vi "Get CTRL Area.vi"(6 "SizeOffset (16)":u32=16, 8 "error in (no error)":errorcluster, 9 "Pane in":refnum<vi>, 11 "Control in":refnum<vi>) -> (0 "error out":errorcluster, 1 "Pane out":refnum<vi>, 2 "InsideTheUI":bool, 3 "Control out":refnum<vi>, 5 "CTRL Area":T1)   [LabVIEW 2019, in "Language Editor.lvlib"]
doc: "- - -\nCopyright (c) 2026, Merecs Engineering GmbH"
uses:
  Language Editor.lvlib
panel:
  # "Connector Pane"
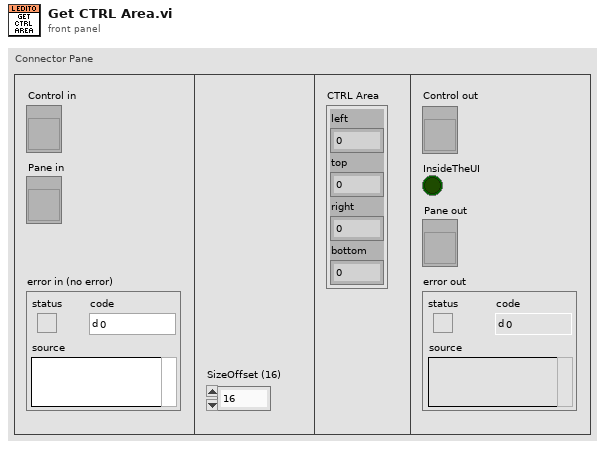
[diagram p1: front panel]
types:
  T1 = cluster{"left":i16, "top":i16, "right":i16, "bottom":i16}
  T2 = typedef "LVPositionTypeDef.ctl" = cluster{"Left":i32, "Top":i32}
  T3 = typedef "LVBoundsTypeDef.ctl" = cluster{"Width":u32, "Height":u32}
  T4 = typedef "LVRectTypeDef.ctl" = cluster{"Left":i16, "Top":i16, "Right":i16, "Bottom":i16}
  T5 = typedef "LVPointTypeDef.ctl" = cluster{"Horizontal":i16, "Vertical":i16}
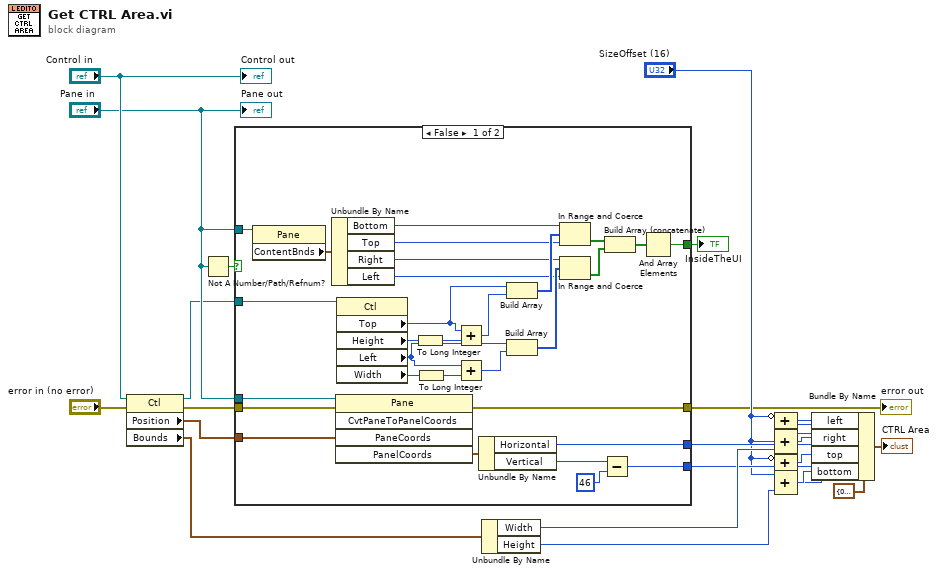
[diagram p0: block diagram]
diagram:
  n1 = property class="Ctl"(reference="Control in", error in="error in (no error)") -> (reference out=w2:refnum<vi>, error out=w10:errorcluster, "Position"=w21:T2, "Bounds"=w9:T3)
  n2 = Not A Number/Path/Refnum?(number/path/refnum="Pane in") -> (NaN/Path/Refnum?=w4:bool)
  n3 = case shown="False" w4 {
    tunnel: w21 -> [w49 _]
    tunnel: "Pane in" -> [w46 _]
    tunnel: w10 -> [w45 w52]
    tunnel: [w44 _] -> w8
    tunnel: [w43 _] -> w7
    tunnel: [w42 w52] -> w5
    tunnel: "Pane in" -> [w22 _]
    tunnel: w2 -> [w37 _]
    tunnel: [w31 _] -> w1
    frame False {
      n4 = property class="Pane"(reference=w22) -> ("ContentBnds"=w27:T4)  [unwired: 1 in, 2 out]
      n5 = Unbundle By Name(w27) -> ("Bottom"=w26:i16, "Top"=w25:i16, "Right"=w24:i16, "Left"=w23:i16)
      n6 = invoke class="Pane" method="CvtPaneToPanelCoords"(reference=w46, error in=w45, "PaneCoords"=w49) -> (error out=w42:errorcluster, "PanelCoords"=w50:T5)  [unwired: 2 in, 3 out]
      n7 = property class="Ctl"(reference=w37) -> ("Top"=w35:i32, "Height"=w38:u32, "Left"=w30:i32, "Width"=w39:u32)  [unwired: 1 in, 2 out]
      n8 = To Long Integer(number=w38) -> (32bit integer=w41:i32)
      n9 = To Long Integer(number=w39) -> (32bit integer=w40:i32)
      n10 = Add(x=w35, y=w41) -> (x+y=w36:i32)
      n11 = Add(x=w30, y=w40) -> (x+y=w29:i32)
      n12 = Unbundle By Name(w50) -> ("Horizontal"=w44:i16, "Vertical"=w47:i16)
      n13 = Build Array(w35, w36) -> (w51:i32[])
      n14 = Build Array(w30, w29) -> (w28:i32[])
      n15 = In Range and Coerce(upper limit=w26, x=w51, lower limit=w25) -> (In Range?=w34:bool[])  [unwired: 1 out]
      n16 = In Range and Coerce(upper limit=w24, x=w28, lower limit=w23) -> (In Range?=w33:bool[])  [unwired: 1 out]
      n17 = Subtract(x=w47, y=i16 46 ("value")) -> (x-y=w43:i16)
      n18 = Build Array (concatenate)(w34, w33) -> (w32:bool[])
      n19 = And Array Elements(Boolean array=w32) -> (logical AND=w31:bool)
    }
    frame True {
    }
  }
  "error out" <- w5
  "InsideTheUI" <- w1
  n20 = Unbundle By Name(w9) -> ("Width"=w17:u32, "Height"=w20:u32)
  n21 = Compound Arithmetic op=ADD(invert "SizeOffset (16)", w8) -> (w15:u32)
  n22 = Compound Arithmetic op=ADD(w8, "SizeOffset (16)", w17) -> (w18:u32)
  n23 = Compound Arithmetic op=ADD(invert "SizeOffset (16)", w7) -> (w16:u32)
  n24 = Compound Arithmetic op=ADD("SizeOffset (16)", w7, w20) -> (w19:u32)
  n25 = Bundle By Name(cluster=T1 {"left"=0, "top"=0, "right"=0, "bottom"=0} ("CTRL Area"), "left"=w15, "right"=w18, "top"=w16, "bottom"=w19) -> (→"CTRL Area":T1)
  "Control out" <- "Control in"
  "Pane out" <- "Pane in"
